vi "Convert RPM to Analog Voltage.vi"(11 "Write to AO":dbl) -> (3 "Numeric":dbl)   [LabVIEW 2021]
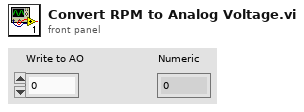
[diagram p1: front panel]
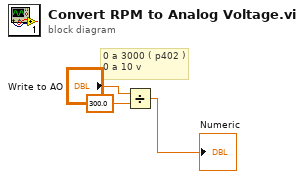
[diagram p0: block diagram]
diagram:
  # "0 a 3000 ( p402 )\n0 a 10 v"
  n1 = Divide(x="Write to AO", y=300.0) -> (x/y=→"Numeric":dbl)
